vi "Get RemIO Read Scaling Factor.vi"(8 "error in (no error)":errorcluster, 10 "11102 in":refnum<class "11102.lvclass">, 11 "Node Ptr In":T1 format="%.0x") -> (0 "error out":errorcluster, 1 "Scaling Factors":dbl[](array[numeric]), 2 "11102 out":refnum<class "11102.lvclass">, 3 "Node Ptr Out":T1 format="%.0x", 5 "Per Channel?":bool)   [LabVIEW 2020, in "Modules.lvlib" / "11102.lvclass"]
doc: "This VI Returns the scaling factors for REM IO Input Modules"
uses:
  11102.lvclass
  <vilib>/NI VeriStand/Custom Device API/Custom Device Item Ref.ctl
  11102.lvclass/11102.ctl
  8565608f-3320-4898-8580-f5a75b88424c.vi
  RemIO Module/Get RemIO Library Path.vi
  <vilib>/NI VeriStand/Custom Device API/Custom Device API.lvlib
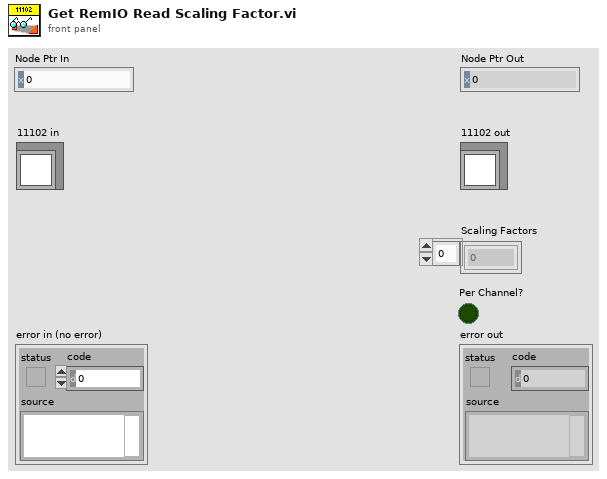
[diagram p1: front panel]
types:
  T1 = typedef "Custom Device API.lvlib/Custom Device Item Ref.ctl" = u64
  T2 = typedef "NI ECAT Remote IO.lvlib/channul number REM-11102.ctl" = u8
  T3 = typedef "NI ECAT Remote IO.lvlib/input filter time REM-11102.ctl" = u8
  T4 = typedef "NI ECAT Remote IO.lvlib/mean-value REM-11102.ctl" = u8
  T5 = typedef "NI ECAT Remote IO.lvlib/measuring range REM-11102.ctl" = u8
  T6 = cluster{"channel number":T2, "input filter time":T3, "mean-value":T4, "measuring range":T5}[]
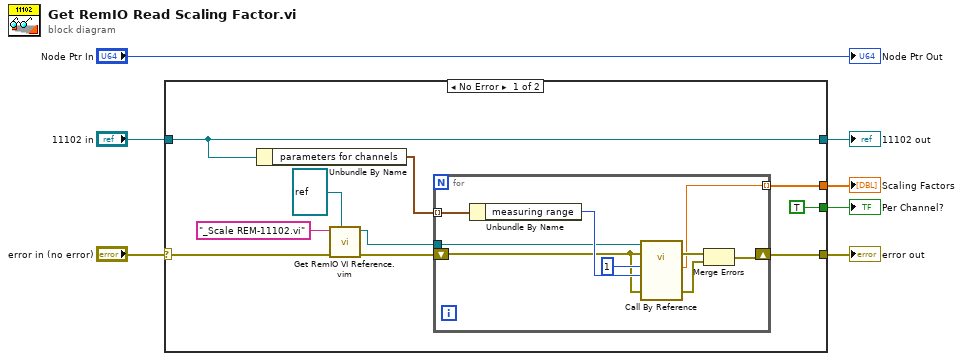
[diagram p0: block diagram]
diagram:
  n1 = case shown="No Error" "error in (no error)" {
    selector: "error in (no error)" -> [w12 w28]
    tunnel: [w16 w28] -> w6
    tunnel: [w15 w27] -> w3
    tunnel: "11102 in" -> [w15 w27]
    tunnel: [TRUE _] -> w2
    tunnel: [w13 _] -> w1
    frame No Error {
      n2 = Unbundle By Name(w15) -> ("parameters for channels"=w14:T6)
      n3 = call "Get RemIO VI Reference.vim"("name or relative path"="_Scale REM-11102.vi", "error in (no error)"=w12, "type specifier VI Refnum (for type only)"=refnum<vi> refnum) -> ("vi reference"=w8:refnum<vi>, "error out"=w11:errorcluster)  [unwired: 6 in]
      n4 = for {
        shift-right: [w21] -> w16
        shift-left: w11 -> [w19]
        tunnel: w14 -> [w26] mode=indexing
        tunnel: [w20] -> w13 mode=indexing
        tunnel: w8 -> [w18]
        n5 = Unbundle By Name(w26) -> ("measuring range"=w22:T5)
        n6 = call-by-ref "?"(reference=w18, error in=w19, 8:"error in (no error)"=w19, "measuring range"=w22, "raw data"=u16 1) -> (error out=w24:errorcluster, 0:"error out"=w25:errorcluster, "scaled data"=w20:dbl)  [unwired: 7 in, 1 out]
        n7 = Merge Errors(w24, w25) -> (w21:errorcluster)
      }
    }
    frame Error {
    }
  }
  "error out" <- w6
  "11102 out" <- w3
  "Scaling Factors" <- w1
  "Per Channel?" <- w2
  "Node Ptr Out" <- "Node Ptr In"
